vi "init.vi"(8 "error in":errorcluster, 10 "TBM module configuration in":refnum<class "TBM module configuration.lvclass">, 11 "TDMS datalogger runtime in":refnum<class "TDMS datalogger runtime.lvclass">) -> (0 "error out":errorcluster, 1 "data allocations":T1, 2 "execution settings":T4, 3 "TDMS datalogger runtime out":refnum<class "TDMS datalogger runtime.lvclass">)   [LabVIEW 2015, in "TDMS datalogger runtime.lvclass"]
doc: "Provides an interface for initializing a module at runtime. While this interface performs no operations, a child should provide an override which may open any necessary references or sessions, allocate necessary memory, and perform any final configuration validataion before providing the full configuration <b>execution data</b> to the calling process."
uses:
  TDMS datalogger runtime.lvclass
  <vilib>/NI/Tag Bus Module Framework/module configuration/TBM module configuration.lvclass
  <vilib>/NI/Tag Bus Module Framework/runtime/execution settings.ctl
  <vilib>/NI/Tag Bus Module Framework/channel/data tables.ctl
  <vilib>/NI/Tag Bus/dictionary/data dictionary.lvclass
  <vilib>/NI/Tag Bus/dictionary table pair.ctl
  <vilib>/NI/Tag Bus/table/data table.ctl
  configuration/TDMS datalogger configuration.lvclass
  message to background process.ctl
  control enum.ctl
  response from background process.ctl
  response enum.ctl
  configuration/TDMS datalogger configuration.lvclass/TDMS datalogger configuration.ctl
  TDMS datalogger runtime.lvclass/TDMS datalogger runtime.ctl
  configuration/Read add enable channel.vi
  configuration/Read queue size.vi
  configuration/Read log directory.vi
  configuration/Read backup directory.vi
  configuration/Read scans per write.vi
  configuration/Read log name.vi
  configuration/Read logrotate_options.vi
  <vilib>/NI/Tag Bus Module Framework/channel/TBM channel.lvclass
  <vilib>/NI/Tag Bus Module Framework/runtime/TBM module execution interface.lvclass
  <vilib>/NI/Tag Bus/table/data table.lvlib
  <vilib>/NI/LogRotate/LogRotate.lvclass
  <vilib>/NI/Tag Bus/tag bus.lvlib
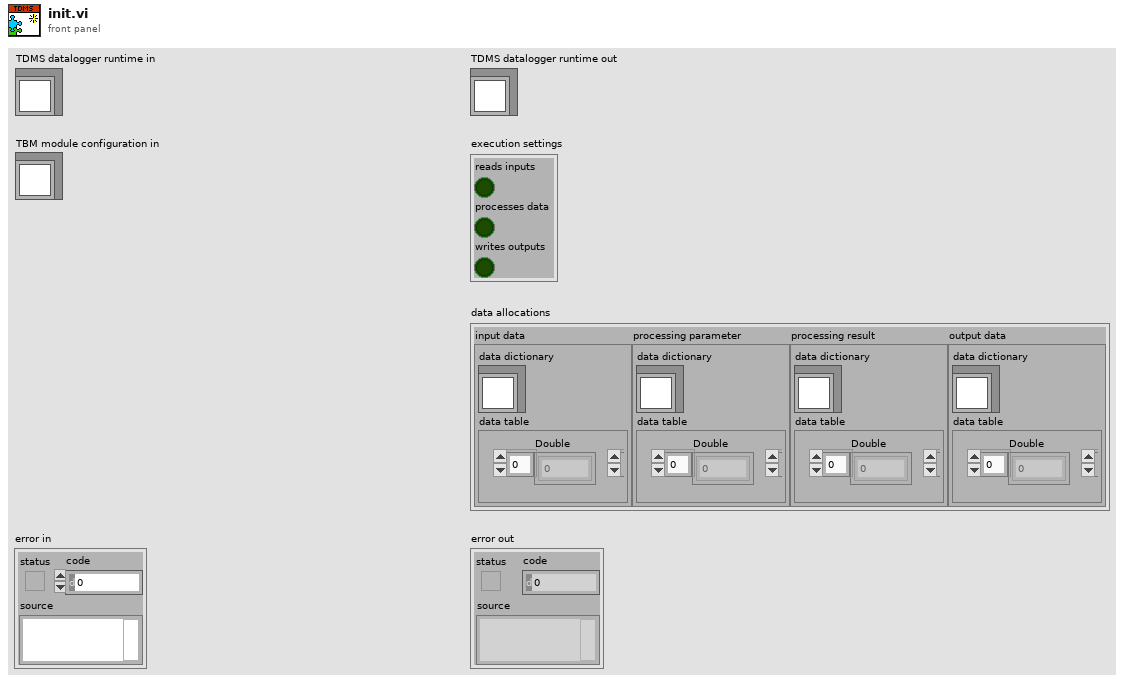
[diagram p1: front panel]
types:
  T1 = typedef "TBM channel.lvclass/data tables.ctl" = cluster{"input data":T2, "processing parameter":T2, "processing result":T2, "output data":T2}
  T2 = typedef "tag bus.lvlib/dictionary table pair.ctl" = cluster{"data dictionary":refnum<class "data dictionary.lvclass">, "data table":T3}
  T3 = typedef "tag bus.lvlib/data table.lvlib/data table.ctl" = cluster{"Double":dbl[], "Single":sgl[], "I64":i64[], "I32":i32[], "I16":i16[], "I8":i8[], "U64":u64[], "U32":u32[], "U16":u16[], "U8":u8[], "Boolean":bool[], "String":string[], "Array of Double":cluster{"DBL Array":dbl[]}[], "Array of Single":cluster{"SGL Array":sgl[]}[], "Array of I64":cluster{"I64 Array":i64[]}[], "Array of I32":cluster{"I32 Array":i32[]}[], "Array of I16":cluster{"I16 Array":i16[]}[], "Array of I8":cluster{"I8 Array":i8[]}[], "Array of U64":cluster{"U64 Array":u64[]}[], "Array of U32":cluster{"U32 Array":u32[]}[], "Array of U16":cluster{"U16 Array":u16[]}[], "Array of U8":cluster{"U8 Array":u8[]}[], "Array of Boolean":cluster{"Boolean Array":bool[]}[], "Array of String":cluster{"String Array":string[]}[]}
  T4 = typedef "TBM module execution interface.lvclass/execution settings.ctl" = cluster{"reads inputs":bool, "processes data":bool, "writes outputs":bool}
  T5 = cluster{"read mode":enum16{"polling", "blocking"}, "write mode":enum16{"polling", "blocking"}}
  T6 = typedef "TDMS datalogger runtime.lvclass/response from background process.ctl" = cluster{"response enum":T7, "datapack":refnum<data-value>, "error code":i32}
  T7 = typedef "TDMS datalogger runtime.lvclass/response enum.ctl" = enum16{"exit", "return buffer", "error"}
  T8 = typedef "TDMS datalogger runtime.lvclass/message to background process.ctl" = cluster{"control enum":T9, "datapack":refnum<data-value>, "Time Stamp":timestamp}
  T9 = typedef "TDMS datalogger runtime.lvclass/control enum.ctl" = enum16{"exit", "output data"}
  T10 = typedef "tag bus.lvlib/tag descriptor.lvclass/Data Type.ctl" = enum16{"Double", "Single", "I64", "I32", "I16", "I8", "U64", "U32", "U16", "U8", "Boolean", "String", "Array of Double", "Array of Single", "Array of I64", "Array of I32", "Array of I16", "Array of I8", "Array of U64", "Array of U32", "Array of U16", "Array of U8", "Array of Boolean", "Array of String"}
  T11 = typedef "LogRotate.lvclass/options.ctl" = cluster{"max file size (bytes)":i64, "rotate count":u32, "max age (days)":dbl, "No archive dir":bool, "Archive dir":path}
  T12 = typedef "tag bus.lvlib/data dictionary.lvclass/full data dictionary.ctl" = cluster{"Double":string[], "Single":string[], "I64":string[], "I32":string[], "I16":string[], "I8":string[], "U64":string[], "U32":string[], "U16":string[], "U8":string[], "Boolean":string[], "String":string[], "Array of Double":string[], "Array of Single":string[], "Array of I64":string[], "Array of I32":string[], "Array of I16":string[], "Array of I8":string[], "Array of U64":string[], "Array of U32":string[], "Array of U16":string[], "Array of U8":string[], "Array of Boolean":string[], "Array of String":string[]}
  T13 = typedef "tag bus.lvlib/data table.lvlib/allocation specification.ctl" = cluster{"data type":T10, "size":i32}
  T14 = typedef "TDMS datalogger runtime.lvclass/data cache.ctl" = cluster{"timestamps":timestamp[], "Double":dbl[][], "Single":sgl[][], "I64":i64[][], "I32":i32[][], "I16":i16[][], "I8":i8[][], "U64":u64[][], "U32":u32[][], "U16":u16[][], "U8":u8[][], "Boolean":bool[][]}
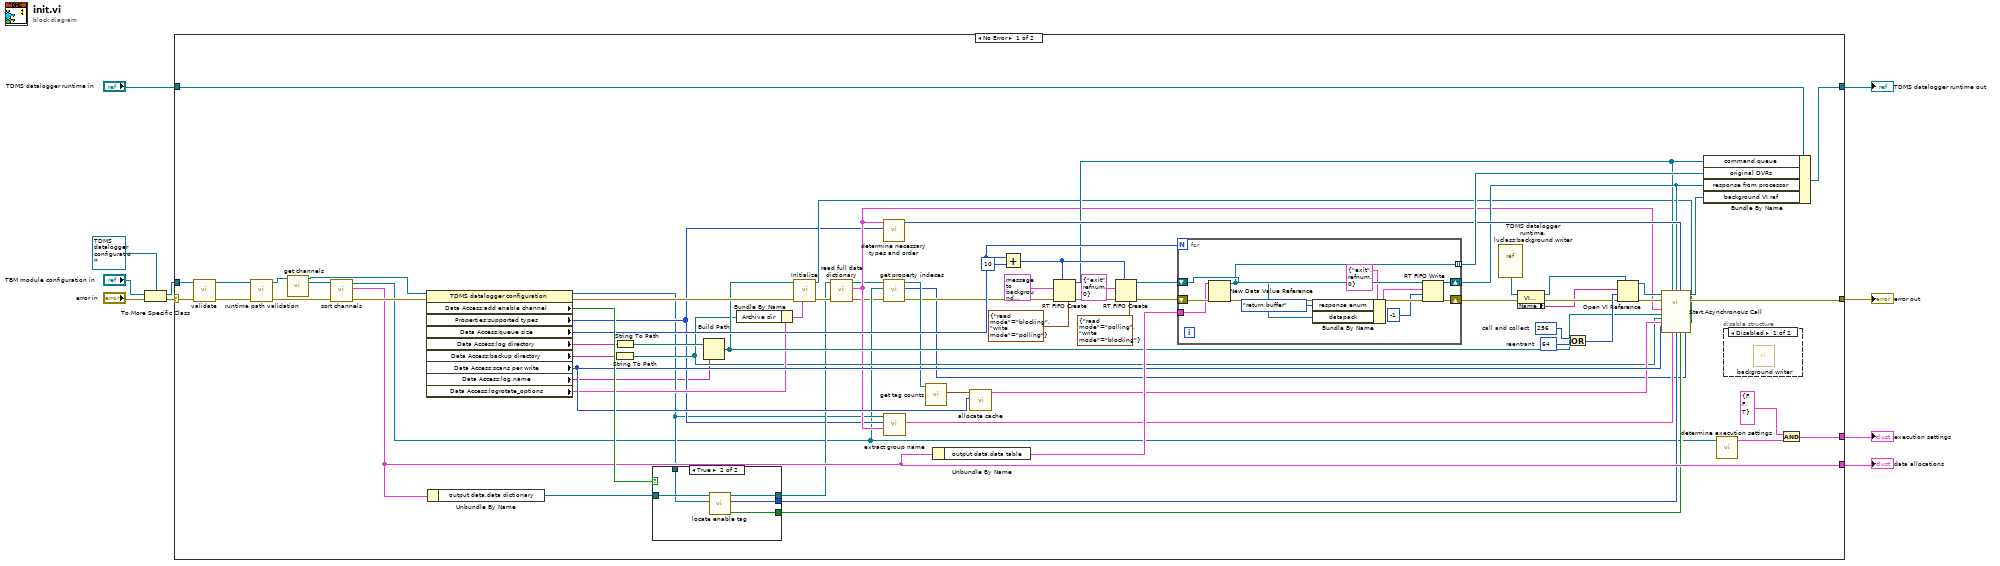
[diagram p0: block diagram]
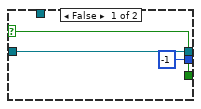
[diagram p2: hidden frame]
diagram:
  n1 = To More Specific Class(target class=refnum<class "TDMS datalogger configuration.lvclass"> refnum ("Synchronous module configuration"), reference="TBM module configuration in", error in="error in") -> (specific class reference=w9:refnum<class "TDMS datalogger configuration.lvclass">, error out=w10:errorcluster)
  n2 = case shown="No Error" w10 {
    selector: w10 -> [w78 w101]
    tunnel: w9 -> [w77 _]
    tunnel: "TDMS datalogger runtime in" -> [w76 w102]
    tunnel: [w75 w102] -> w4
    tunnel: [w64 w101] -> w3
    tunnel: [w62 _] -> w1
    tunnel: [w74 _] -> w2
    frame No Error {
      w69 = 64  # reentrant
      w68 = 256  # call and collect
      n3 = call-dynamic "validate.vi"("error in"=w78, "TDMS datalogger configuration in"=w77) -> ("error out"=w79:errorcluster, "TDMS datalogger configuration out"=w59:refnum<class "TDMS datalogger configuration.lvclass">)  [unwired: 8 in]
      n4 = call "runtime path validation.vi"("error in"=w79, "TDMS datalogger configuration in"=w59) -> ("error out"=w60:errorcluster, "TDMS datalogger configuration out"=w58:refnum<class "TDMS datalogger configuration.lvclass">)  [unwired: 8 in]
      n5 = call-dynamic "get channels.vi"("module configuration in"=w58) -> ("channels"=w18:refnum<class "TBM channel.lvclass">[], "module configuration out"=w57:refnum<class "TDMS datalogger configuration.lvclass">)  [unwired: 9 in]
      n6 = call <vilib>:"sort channels.vi"("error in"=w60, "channels in"=w18) -> ("error out"=w81:errorcluster, "data allocations"=w62:T1, "channels out"=w14:refnum<class "TBM channel.lvclass">[])  [unwired: 7 in]
      n7 = property class="TDMS datalogger configuration"(reference=w57, error in=w81) -> (reference out=w21:refnum<class "TDMS datalogger configuration.lvclass">, error out=w31:errorcluster, "Data Access:add enable channel"=w63:bool, "Properties:supported types"=w22:T10[], "Data Access:queue size"=w47:u16, "Data Access:log directory"=w34:string, "Data Access:backup directory"=w33:string, "Data Access:scans per write"=w39:u16, "Data Access:log name"=w19:string, "Data Access:logrotate_options"=w29:T11)
      n8 = Unbundle By Name(w62) -> ("output data.data dictionary"=w17:refnum<class "data dictionary.lvclass">)
      n9 = String To Path(string=w33) -> (path=w28:path)
      n10 = String To Path(string=w34) -> (path=w32:path)
      n11 = case shown="True" w63 {
        selector: w63 -> [w84 _]
        tunnel: w17 -> [w83 w89]
        tunnel: [w83 w88] -> w24
        tunnel: [w84 w86] -> w41
        tunnel: [-1 ("index") w87] -> w40
        tunnel: w21 -> [_ w85]
        frame False {
        }
        frame True {
          n12 = call "locate enable tag.vi"("TDMS datalogger configuration"=w85, "data dictionary in"=w89) -> ("found?"=w86:bool, "index"=w87:i32, "data dictionary out"=w88:refnum<class "data dictionary.lvclass">)  [unwired: 7 in]
        }
      }
      n13 = Build Path(base path=w32, name or relative path=w19) -> (appended path=w30:path)
      n14 = Bundle By Name(cluster=w29, "Archive dir"=w28) -> (w27:T11)
      n15 = call <vilib>:"Initialize.vi"("Options"=w27, "error in (no error)"=w31, "Log File Path"=w30) -> ("error out"=w26:errorcluster, "LogRotate"=w25:refnum<class "LogRotate.lvclass">)  [unwired: 7 in]
      n16 = call <vilib>:"read full data dictionary.vi"("error in"=w26, "data dictionary in"=w24) -> ("error out"=w13:errorcluster, "dictionary"=w23:T12, "data dictionary out"=w16:refnum<class "data dictionary.lvclass">)  [unwired: 7 in]
      n17 = call "determine necessary types and order.vi"("supported types"=w22, "dictionary"=w23) -> ("output type order"=w37:T10[])  [unwired: 9 in]
      n18 = call "get property indeces.vi"("error in"=w13, "channels"=w14, "data dictionary in"=w16) -> ("error out"=w12:errorcluster, "File Property Indeces"=w11:i32[], "data dictionary out"=w15:refnum<class "data dictionary.lvclass">)  [unwired: 6 in]
      n19 = call "extract group name.vi"("dictionary"=w23, "supported types"=w22, "TDMS datalogger configuration in"=w21) -> ("dictionary group names"=w20:T12)  [unwired: 8 in]
      n20 = call <vilib>:"get tag counts.vi"("data dictionary in"=w15) -> ("counts"=w72:T13[])  [unwired: 9 in, 1 out]
      n21 = Unbundle By Name(w62) -> ("output data.data table"=w56:T3)
      n22 = call "allocate cache.vi"("scans per write"=w39, "counts"=w72) -> ("cache allocation"=w38:T14)  [unwired: 9 in]
      n23 = Add(x=w47, y=u16 10) -> (x+y=w45:u16)
      n24 = RT FIFO Create(1:T8 {"control enum"=enum."exit", "datapack"=refnum, "Time Stamp"=timestamp(0 s since 1904-01-01)} ("message"), 3:w12, 4:w45, 7:T5 {"read mode"=enum."blocking", "write mode"=enum."polling"} ("r/w modes (polling,polling)")) -> (8:w35:refnum<k33>, 11:w55:errorcluster)  [unwired: 4 in, 1 out]
      n25 = RT FIFO Create(1:T6 {"response enum"=enum."exit", "datapack"=refnum, "error code"=0} ("message"), 3:w55, 4:w45, 7:T5 {"read mode"=enum."polling", "write mode"=enum."blocking"} ("r/w modes (polling,polling)")) -> (8:w48:refnum<k33>, 11:w52:errorcluster)  [unwired: 4 in, 1 out]
      n26 = for {
        N: w47 -> [_]
        shift-right: [w97] -> w65
        shift-left: w52 -> [w100]
        tunnel: w56 -> [w99]
        tunnel: [w91] -> w49 mode=indexing
        shift-right: [w96] -> w36
        shift-left: w48 -> [w95]
        n27 = New Data Value Reference(data value=w99, error in=w100) -> (data value reference=w91:refnum<data-value>, error out=w98:errorcluster)
        n28 = Bundle By Name(cluster=T6 {"response enum"=enum."exit", "datapack"=refnum, "error code"=0} ("element"), "response enum"=response_enum."return buffer", "datapack"=w91) -> (w92:T6)
        n29 = RT FIFO Write(0:w95, 1:w92, 2:-1 ("timeout in ms (0)"), 3:w98) -> (8:w96:refnum<k33>, 11:w97:errorcluster)  [unwired: 1 in, 2 out]
      }
      n30 = vi-ref "TDMS datalogger runtime.lvclass:background writer.vi"() -> (w44:refnum<vi>)
      n31 = property class="VI (strict)"(reference=w44, error in=w65) -> (reference out=w43:refnum<vi>, error out=w67:errorcluster, "Name"=w66:string)
      n32 = Or(x=w68, y=w69) -> (x .or. y?=w70:i32)
      n33 = Open VI Reference(type specifier VI Refnum (for type only)=w43, vi path=w66, options=w70, error in (no error)=w67) -> (vi reference=w42:refnum<vi>, error out=w71:errorcluster)  [unwired: 2 in]
      n34 = call-by-ref "Start Asynchronous Call"(reference=w42, error in=w71, "dictionary"=w23, "command queue"=w35, "response from processor"=w36, "output type order"=w37, "File Property Indeces"=w11, "logging path"=w30, "backup directory"=w28, "cache allocation"=w38, "LogRotate"=w25, "scans per write"=w39, "dictionary group names"=w20, "enable channel (bool)"=w40, "has enable channel"=w41) -> (reference out=w61:refnum<vi>, error out=w64:errorcluster)  [unwired: 2 in, 1 out]
      n35 = Bundle By Name(cluster=w76, "command queue"=w35, "original DVRs"=w49, "response from processor"=w36, "background VI ref"=w61) -> (w75:refnum<class "TDMS datalogger runtime.lvclass">)
      n36 = call <vilib>:"determine execution settings.vi"("channels"=w14) -> ("execution settings"=w80:T4)  [unwired: 10 in]
      n37 = disable-structure shown="Disabled" {
        frame Disabled {
          n38 = call "background writer.vi"() -> ()  [unwired: 15 in, 1 out]
        }
        frame Enabled {
        }
      }
      n39 = And(x=T4 {"reads inputs"=FALSE, "processes data"=FALSE, "writes outputs"=TRUE}, y=w80) -> (x .and. y?=w74:T4)
    }
    frame Error {
    }
  }
  "error out" <- w3
  "TDMS datalogger runtime out" <- w4
  "execution settings" <- w2
  "data allocations" <- w1
